vi "linked-ignore.vi"(11 "error in":errorcluster) -> (15 "error out":errorcluster)   [LabVIEW 2024]
doc: "Data-only fixture for object-scoped path-usage ignores. No file operations are performed."
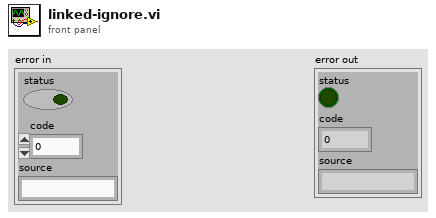
[diagram p1: front panel]
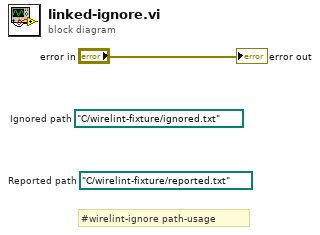
[diagram p0: block diagram]
diagram:
  (unwired) path "C:/wirelint-fixture/reported.txt"  # Reported path
  (unwired) path "C:/wirelint-fixture/ignored.txt"  # Ignored path
  # "#wirelint-ignore path-usage"
  "error out" <- "error in"
